vi "Handle Error.vi"(8 "error in (no error)":errorcluster, 11 "CIFPlugin in":refnum<class "CAN_Writer_NIXNET_Plugin.lvclass">) -> (0 "error out":errorcluster, 3 "CIFPlugin out":refnum<class "CAN_Writer_NIXNET_Plugin.lvclass">)   [LabVIEW 2021, in "CAN_Writer_NIXNET_Plugin.lvclass"]
uses:
  CAN_Writer_NIXNET_Plugin.lvclass
  CAN_Writer_NIXNET_Plugin.lvclass/CAN_Writer_NIXNET_Plugin.ctl
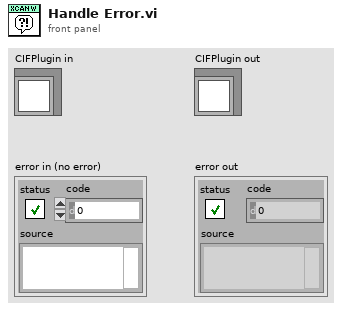
[diagram p1: front panel]
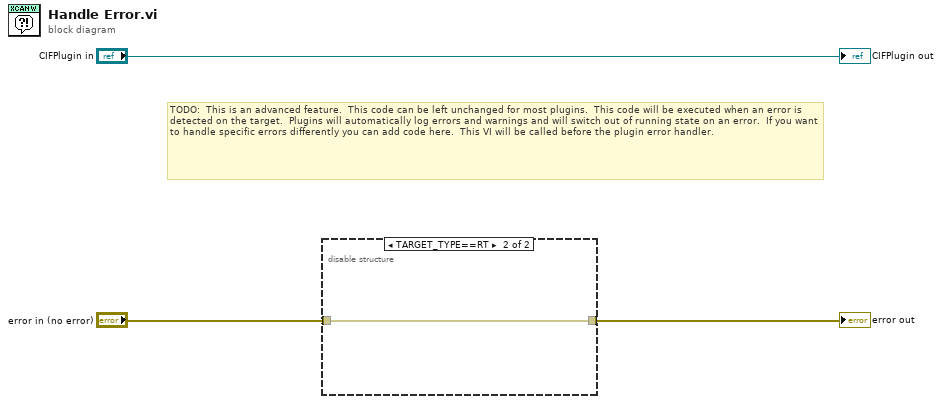
[diagram p0: block diagram]
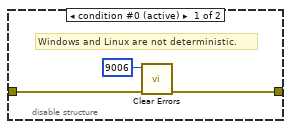
[diagram p2: hidden frame]
diagram:
  # "TODO:  This is an advanced feature.  This code can be left unchanged for most plugins.  This code will be executed when an error is detected on the target.  Plugins will automatically log errors and warnings and will switch out of running state on an error.  If you want to handle specific errors differently you can add code here.  This VI will be called before the plugin error handler."
  n1 = disable-structure shown="TARGET_TYPE==RT" {
    disable-tunnel: "error in (no error)" -> [w6 w7]
    disable-tunnel: [w5 w7] -> w1
    frame condition #0 (active) {
      # "Windows and Linux are not deterministic."
      n2 = call <vilib>:"Clear Errors.vi"("error in (no error)"=w6, "specific error code to clear (0: all)"=9006) -> ("error out"=w5:errorcluster)  [unwired: 4 in, 1 out]
    }
    frame condition #1 {
    }
  }
  "error out" <- w1
  "CIFPlugin out" <- "CIFPlugin in"
